vi "Interface.vi"() -> ()   [LabVIEW 2019, in "Socket Auto Connect.lvclass"]
uses:
  Socket Auto Connect.lvclass
  Robot/Universal Robot/Universal Robot.lvclass
  C:/_Code/Development/Sub-Zero Functional Test/standard hardware/Universal Robots/UR LabVIEW Interface/Classes/Application/Application Interfaces/Application Interface/Application Interface.lvclass
  Socket Auto Connect.lvclass/Socket Auto Connect.ctl
  Client Interfaces/Socket Communication/Socket Communication.lvclass
  Application.lvclass
  Application Interface/Application Interface.lvclass
panel:
  out "connected":bool
  out "running":bool
  out "Data Viewer":string
  in  "interface":refnum<class "Socket Auto Connect.lvclass">
  in  "robot":refnum<class "Universal Robot.lvclass">
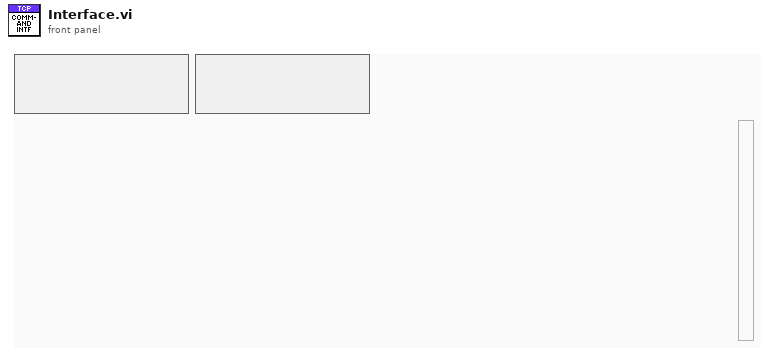
[diagram p1: front panel]
types:
  T1 = typedef "Application.lvclass/FrontPanelControls.ctl" = cluster{"Operation Interface":refnum<vi>, "Program Interface":refnum<vi>, "Command Interface":refnum<vi>, "Socket Interface":refnum<vi>, "Error Interface":refnum<vi>}
  T2 = typedef "Universal Robot.lvclass/ProgramStatus.ctl" = cluster{"Loaded Program":string, "Valid Program":bool, "Program State":T3, "Running":bool}
  T3 = typedef "Universal Robot.lvclass/ProgramState.ctl" = enum16{"STOPPED", "PLAYING", "PAUSE"}
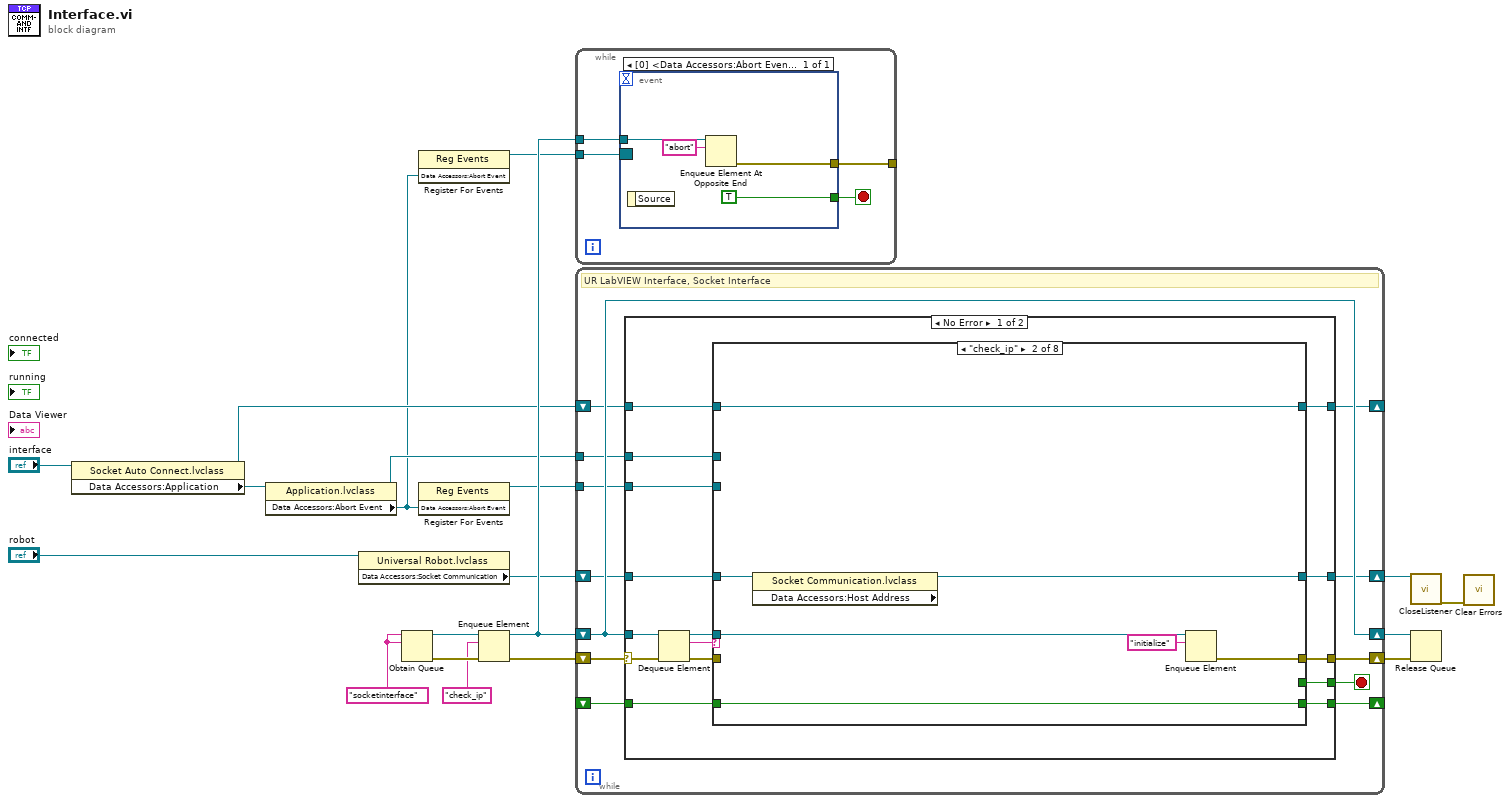
[diagram p0: block diagram]
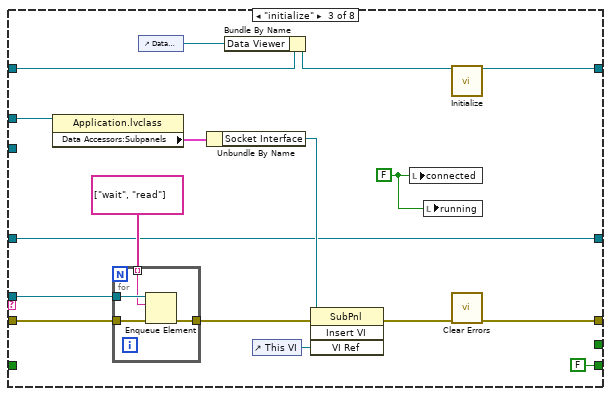
[diagram p3: hidden frame]
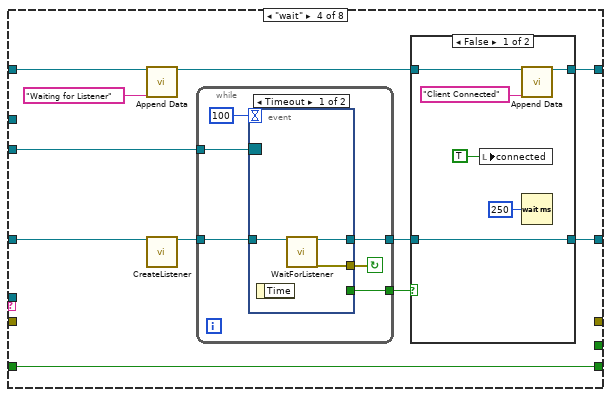
[diagram p4: hidden frame]
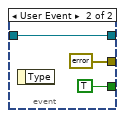
[diagram p6: hidden frame]
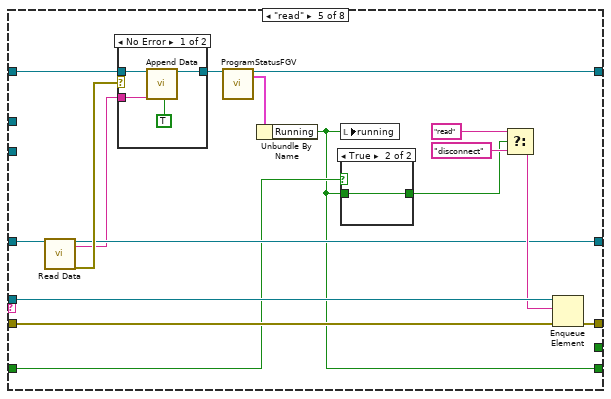
[diagram p7: hidden frame]
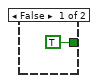
[diagram p8: hidden frame]
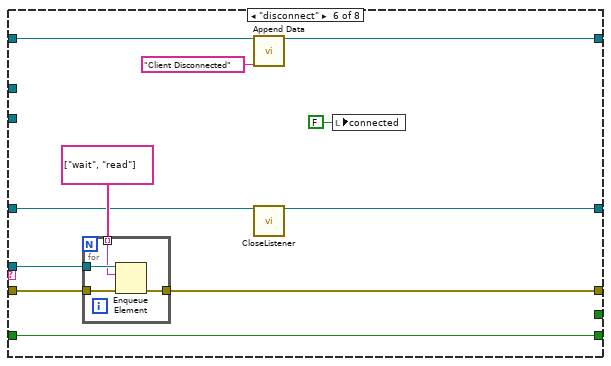
[diagram p10: hidden frame]
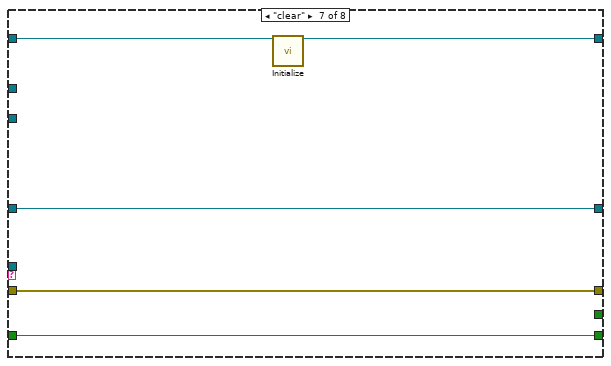
[diagram p11: hidden frame]
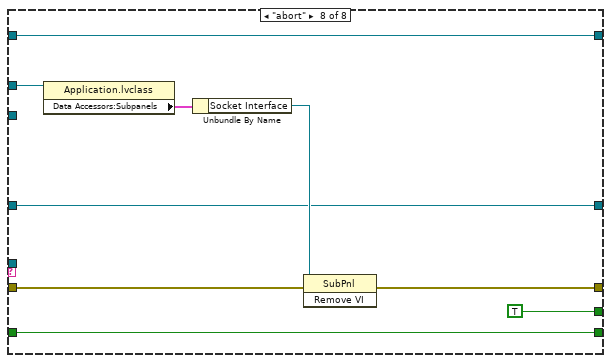
[diagram p12: hidden frame]
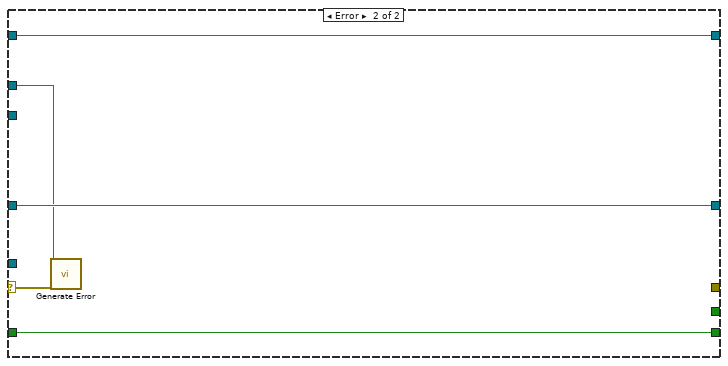
[diagram p13: hidden frame]
diagram:
  w14 = "socketinterface" ("name (unnamed)")
  n1 = property class="Socket Auto Connect.lvclass"(reference="interface") -> (reference out=w9:refnum<class "Socket Auto Connect.lvclass">, "Data Accessors:Application"=w11:refnum<class "Application.lvclass">)  [unwired: 1 in, 1 out]
  n2 = property class="Application.lvclass"(reference=w11) -> (reference out=w8:refnum<class "Application.lvclass">, "Data Accessors:Abort Event"=w3:refnum<user-event>)  [unwired: 1 in, 1 out]
  n3 = property class="Universal Robot.lvclass"(reference="robot") -> ("Data Accessors:Socket Communication"=w6:refnum<class "Socket Communication.lvclass">)  [unwired: 1 in, 2 out]
  n4 = Obtain Queue(name (unnamed)=w14, element data type=w14) -> (queue out=w18:refnum<queue>, error out=w19:errorcluster)  [unwired: 3 in, 1 out]
  n5 = register-events(w3) -> (reference out=w4:refnum<event-registration>)  [unwired: 2 in, 1 out]
  n6 = register-events(w3) -> (reference out=w5:refnum<event-registration>)  [unwired: 2 in, 1 out]
  n7 = Enqueue Element(queue=w18, element="check_ip", error in (no error)=w19) -> (queue out=w15:refnum<queue>, error out=w16:errorcluster)  [unwired: 1 in, 1 out]
  n8 = while {
    tunnel: w15 -> [w23]
    tunnel: w4 -> [w22]
    tunnel: [w21] -> _
    stop <- w20 stop-if-true
    n9 = event shown="[0] <Data Accessors:Abort Event>: User Event" {
      selector: w22 -> [_]
      dyn-events: _ -> [_]
      timeout: _ -> [_]
      tunnel: w23 -> [w27]
      tunnel: [w26] -> w21
      tunnel: [TRUE] -> w20
      event User Event {
        n10 = event-data() -> ()  [unwired: 1 in, 1 out]
        n11 = Enqueue Element At Opposite End(queue=w27, element="abort") -> (error out=w26:errorcluster)  [unwired: 2 in, 2 out]
      }
    }
  }
  n12 = while {
    shift-right: [w37] -> w12
    shift-left: w16 -> [w39]
    shift-right: [w38] -> w13
    shift-left: w15 -> [w38]
    tunnel: w5 -> [w35]
    shift-right: [w33] -> _
    shift-left: w9 -> [w34]
    tunnel: w8 -> [w32]
    shift-right: [w30] -> w2
    shift-left: w6 -> [w31]
    shift-right: [w29] -> _
    shift-left: _ -> [w28]
    stop <- w36 stop-if-true
    # "UR LabVIEW Interface, Socket Interface"
    n13 = case shown="No Error" w39 {
      selector: w39 -> [w53 w172]
      tunnel: w38 -> [w54 _]
      tunnel: [w49 _] -> w37
      tunnel: [w48 _] -> w36
      tunnel: w35 -> [w47 _]
      tunnel: w34 -> [w46 w175]
      tunnel: [w45 w175] -> w33
      tunnel: w32 -> [w44 w171]
      tunnel: w31 -> [w43 w174]
      tunnel: [w42 w174] -> w30
      tunnel: [w41 w173] -> w29
      tunnel: w28 -> [w40 w173]
      frame No Error {
        n14 = Dequeue Element(queue=w54, error in (no error)=w53) -> (queue out=w50:refnum<queue>, element=w51:string, error out=w52:errorcluster)  [unwired: 1 in, 1 out]
        n15 = case shown="\"check_ip\"" w51 {
          tunnel: w52 -> [w58 _ w73 _ w127 w146 w160 w169]
          tunnel: w50 -> [_ w60 w74 _ w128 w147 _ _]
          tunnel: [w58 w61 w68 _ w125 w145 w160 w168] -> w49
          tunnel: [_ _ _ _ _ _ _ TRUE] -> w48
          tunnel: w47 -> [_ _ _ w97 _ _ _ _]
          tunnel: w46 -> [w57 w65 w79 w96 w130 w152 w159 w165]
          tunnel: [w57 w65 w77 w93 w134 w151 w158 w165] -> w45
          tunnel: w44 -> [_ _ w75 _ _ _ _ w164]
          tunnel: w43 -> [w56 w63 w67 w87 w132 w143 w161 w163]
          tunnel: [w56 w62 w67 w90 w122 w142 w161 w163] -> w42
          tunnel: [w55 w64 FALSE ("Running") w89 w119 w144 w157 w162] -> w41
          tunnel: w40 -> [w55 w64 _ w89 w120 w144 w157 w162]
          frame Default {
          }
          frame "check_ip" {
            n16 = property class="Socket Communication.lvclass" props=["Data Accessors:Host Address"](reference=w63) -> (reference out=w62:refnum<class "Socket Communication.lvclass">)  [unwired: 1 in, 2 out]
            n17 = Enqueue Element(queue=w60, element="initialize") -> (error out=w61:errorcluster)  [unwired: 2 in, 2 out]
          }
          frame "initialize" {
            w70 = FALSE ("connected")
            n18 = property class="Application.lvclass"(reference=w75) -> ("Data Accessors:Subpanels"=w81:T1)  [unwired: 1 in, 2 out]
            n19 = for {
              tunnel: w74 -> [w86]
              tunnel: w73 -> [w85]
              tunnel: [w84] -> w72
              tunnel: string[] ["wait", "read"] -> [w83] mode=indexing
              n20 = Enqueue Element(queue=w86, element=w83, error in (no error)=w85) -> (error out=w84:errorcluster)  [unwired: 1 in, 2 out]
            }
            n21 = control-ref of="Data Viewer"() -> (w78:refnum<vi>)
            n22 = Unbundle By Name(w81) -> ("Socket Interface"=w80:refnum<vi>)
            n23 = Bundle By Name(cluster=w79, "Data Viewer"=w78) -> (w76:refnum<class "Socket Auto Connect.lvclass">)
            n24 = control-ref of="This VI"() -> (w82:refnum<vi>)
            n25 = invoke class="SubPnl" method="Insert VI"(reference=w80, error in=w72, "VI Ref"=w82) -> (error out=w69:errorcluster)  [unwired: 1 in, 3 out]
            n26 = local write "connected"(w70) -> ()
            n27 = local write "running"(w70) -> ()
            n28 = call "Initialize.vi"("Socket Auto Connect in"=w76) -> ("Socket Auto Connect out"=w77:refnum<class "Socket Auto Connect.lvclass">)  [unwired: 17 in, 1 out]
            n29 = call <vilib>:"Clear Errors.vi"("error in (no error)"=w69) -> ("error out"=w68:errorcluster)  [unwired: 5 in, 1 out]
          }
          frame "wait" {
            n30 = call "Append Data.vi"("Socket Auto Connect in"=w96, "String to Append"="Waiting for Listener") -> ("Socket Auto Connect out"=w94:refnum<class "Socket Auto Connect.lvclass">)  [unwired: 16 in, 1 out]
            n31 = call "CreateListener.vi"("Socket Listener in"=w87) -> ("Socket Listener out"=w88:refnum<class "Socket Communication.lvclass">)  [unwired: 17 in, 1 out]
            n32 = while {
              tunnel: w88 -> [w111]
              tunnel: w97 -> [w109]
              tunnel: [w107] -> w92
              tunnel: [w106] -> w91
              stop <- w108 continue-if-true
              n33 = event shown="[0] Timeout" {
                selector: w109 -> [_ _]
                dyn-events: _ -> [_ _]
                timeout: 100 -> [_ _]
                tunnel: w111 -> [w114 w116]
                tunnel: [w113 errorcluster {"status"=FALSE, "code"=0, "source"=""} ("error out")] -> w108
                tunnel: [_ TRUE] -> w107
                tunnel: [w112 w116] -> w106
                event Timeout {
                  n34 = event-data() -> ()  [unwired: 1 in, 1 out]
                  n35 = call "WaitForListener.vi"("Socket Listener in"=w114) -> ("Socket Listener out"=w112:refnum<class "Socket Communication.lvclass">, "error out"=w113:errorcluster)  [unwired: 17 in]
                }
                event User Event {
                  n36 = event-data() -> ()  [unwired: 1 in, 1 out]
                }
              }
            }
            n37 = case shown="False" w92 {
              tunnel: w94 -> [w103 w105]
              tunnel: [w102 w105] -> w93
              tunnel: w91 -> [w98 w104]
              tunnel: [w98 w104] -> w90
              frame False {
                n38 = local write "connected"(TRUE ("connected")) -> ()
                n39 = call "Append Data.vi"("Socket Auto Connect in"=w103, "String to Append"="Client Connected") -> ("Socket Auto Connect out"=w102:refnum<class "Socket Auto Connect.lvclass">)  [unwired: 16 in, 1 out]
                n40 = Wait (ms)(milliseconds to wait=u32 250) -> ()  [unwired: 1 out]
              }
              frame True {
              }
            }
          }
          frame "read" {
            n41 = call-dynamic "Read Data.vi"("TCP Socket in"=w132) -> ("TCP Socket out"=w122:refnum<class "Socket Communication.lvclass">, "data"=w121:string, "error out"=w129:errorcluster)  [unwired: 16 in]
            n42 = case shown="No Error" w129 {
              tunnel: [w140 w141] -> w131
              tunnel: w130 -> [w139 w141]
              tunnel: w121 -> [w138 _]
              frame No Error {
                n43 = call "Append Data.vi"("Socket Auto Connect in"=w139, "String to Append"=w138, "Return (T)"=TRUE) -> ("Socket Auto Connect out"=w140:refnum<class "Socket Auto Connect.lvclass">)  [unwired: 15 in, 1 out]
              }
              frame Error {
              }
            }
            n44 = call "ProgramStatusFGV.vi"("Application Interface in"=w131) -> ("Application Interface out"=w134:refnum<class "Socket Auto Connect.lvclass">, "Program Status out"=w133:T2)  [unwired: 16 in, 1 out]
            n45 = Unbundle By Name(w133) -> ("Running"=w119:bool)
            n46 = local write "running"(w119) -> ()
            n47 = case shown="True" w120 {
              tunnel: w119 -> [_ w136]
              tunnel: [TRUE ("Running") w136] -> w118
              frame False {
              }
              frame True {
              }
            }
            n48 = Select(t="read", s=w118, f="disconnect") -> (s? t:f=w124:string)
            n49 = Enqueue Element(queue=w128, element=w124, error in (no error)=w127) -> (error out=w125:errorcluster)  [unwired: 1 in, 2 out]
          }
          frame "disconnect" {
            n50 = for {
              tunnel: w147 -> [w156]
              tunnel: w146 -> [w155]
              tunnel: [w154] -> w145
              tunnel: string[] ["wait", "read"] -> [w153] mode=indexing
              n51 = Enqueue Element(queue=w156, element=w153, error in (no error)=w155) -> (error out=w154:errorcluster)  [unwired: 1 in, 2 out]
            }
            n52 = call "Append Data.vi"("Socket Auto Connect in"=w152, "String to Append"="Client Disconnected") -> ("Socket Auto Connect out"=w151:refnum<class "Socket Auto Connect.lvclass">)  [unwired: 16 in, 1 out]
            n53 = call-dynamic "CloseListener.vi"("TCP Socket in"=w143) -> ("TCP Socket out"=w142:refnum<class "Socket Communication.lvclass">)  [unwired: 17 in, 1 out]
            n54 = local write "connected"(FALSE ("connected")) -> ()
          }
          frame "clear" {
            n55 = call "Initialize.vi"("Socket Auto Connect in"=w159) -> ("Socket Auto Connect out"=w158:refnum<class "Socket Auto Connect.lvclass">)  [unwired: 17 in, 1 out]
          }
          frame "abort" {
            n56 = property class="Application.lvclass"(reference=w164) -> ("Data Accessors:Subpanels"=w167:T1)  [unwired: 1 in, 2 out]
            n57 = Unbundle By Name(w167) -> ("Socket Interface"=w166:refnum<vi>)
            n58 = invoke class="SubPnl" method="Remove VI"(reference=w166, error in=w169) -> (error out=w168:errorcluster)  [unwired: 1 in, 2 out]
          }
        }
      }
      frame Error {
        n59 = call "Generate Error.vi"("Application in"=w171, "error in (no error)"=w172) -> ()  [unwired: 17 in, 1 out]
      }
    }
  }
  n60 = call-dynamic "CloseListener.vi"("TCP Socket in"=w2) -> ("error out"=w1:errorcluster)  [unwired: 17 in, 1 out]
  n61 = Release Queue(queue=w13, error in (no error)=w12) -> ()  [unwired: 1 in, 3 out]
  n62 = call <vilib>:"Clear Errors.vi"("error in (no error)"=w1) -> ()  [unwired: 5 in, 2 out]
